vi "JSON To Control Value.vi"(8 "error in":errorcluster, 9 "JSON":string, 10 "control name":string, 11 "VI reference":refnum<vi>) -> (0 "error out":errorcluster, 3 "value":variant)   [LabVIEW 2020, in "MCP Server.lvlib"]
doc: "Converts the JSON value of one tools/call argument into the data type of the control it is for. The control's current value supplies the type, and JSONtext parses the JSON into exactly that type: numbers of any representation, Booleans, strings, paths, timestamps as ISO 8601 / RFC 3339 strings (\"2026-10-17T12:34:56Z\"), enums by their item names, clusters from objects whose member names are the element labels (a member left out keeps the control's value), and arrays of any number of dimensions and any of these element types. Call VI.vi writes the result to the control. A value that does not fit the type is an error, for example a number for an enum."
uses:
  MCP Server.lvlib
  <vilib>/JDP Science/JSONtext/JSONtext.lvlib
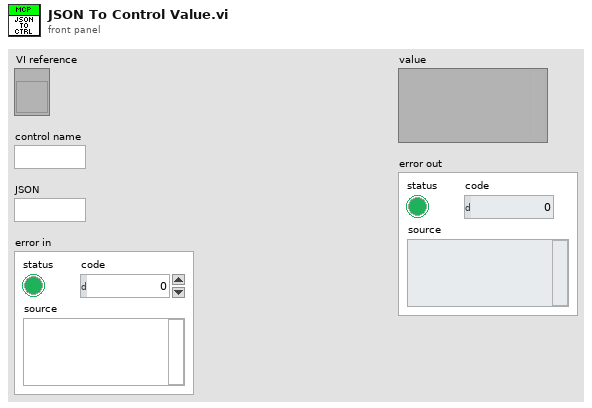
[diagram p1: front panel]
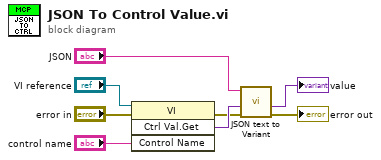
[diagram p0: block diagram]
diagram:
  n1 = invoke class="VI" method="Ctrl Val.Get"(reference="VI reference", error in="error in", "Control Name"="control name") -> (error out=w4:errorcluster, "Get Control Value Variant"=w5:variant)  [unwired: 1 in, 2 out]
  n2 = call <vilib>:"JSON text to Variant.vi"("error in (no error)"=w4, "Data Type"=w5, "JSON"="JSON") -> ("error out"=→"error out":errorcluster, "Variant out"=→"value":variant)  [unwired: 7 in]
